vi "LabVIEW.Service.Create a failed report text from the report array.vi"(8 "error in (no error)":errorcluster caption="Fehler (Eingang, kein Fehler)", 11 "Result[[]]":string[][](array[string])) -> (0 "error out":errorcluster caption="Fehler (Ausgang)", 2 "Passed?":bool, 3 "report text":string)   [LabVIEW 2019]
uses:
  <userlib>/_OpenG.lib/array/array.llb/Search 1D Array (String)__ogtk.vi
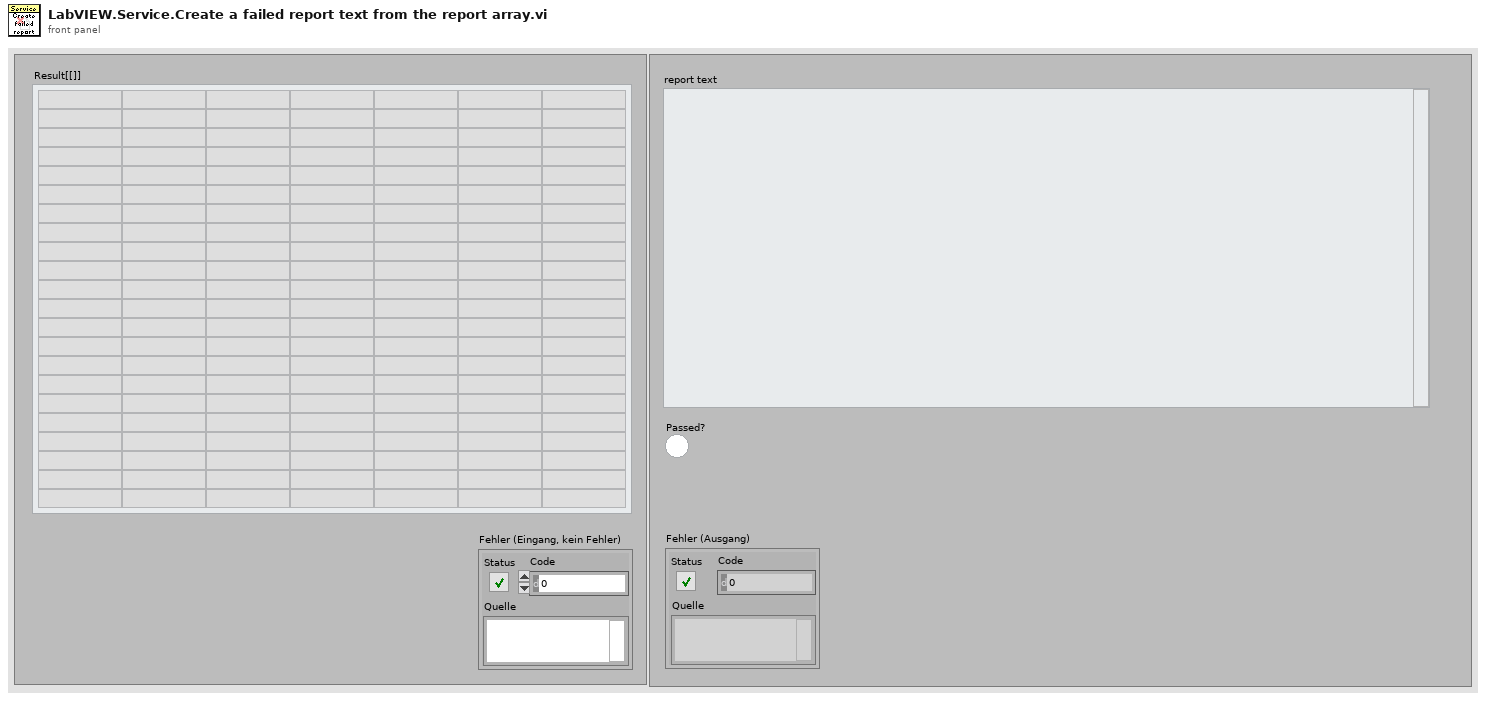
[diagram p1: front panel]
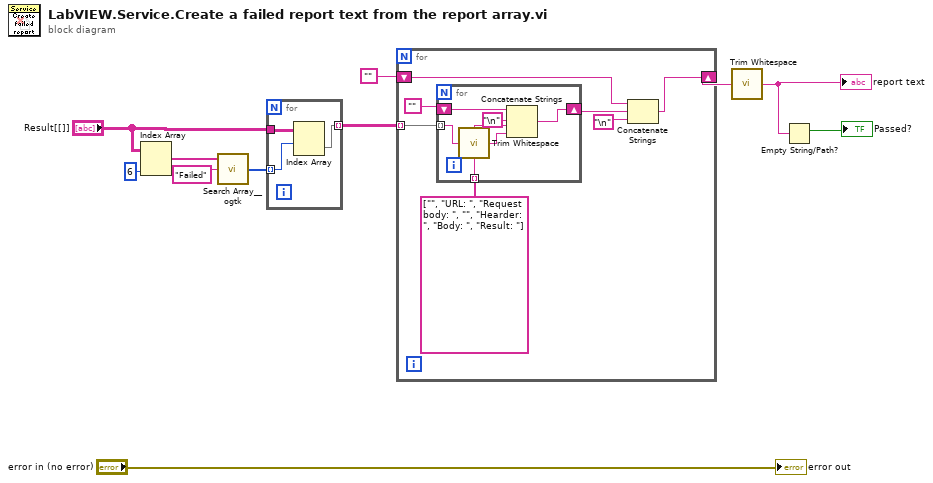
[diagram p0: block diagram]
diagram:
  n1 = Index Array(array="Result[[]]", index (col)=6 ("Deaktivierter Index (Spalte)")) -> (element=w9:string[])  [unwired: 1 in]
  n2 = call-poly <userlib>:"Search Array__ogtk.vi"("Array"=w9, "Element Data"="Failed") -> ("Indices of Elements"=w6:i32[])  [unwired: 7 in]
  n3 = for {
    tunnel: "Result[[]]" -> [w14]
    tunnel: w6 -> [w13] mode=indexing
    tunnel: [w12] -> w5 mode=indexing
    n4 = Index Array(array=w14, index (row)=w13) -> (element=w12:string[])  [unwired: 1 in]
  }
  n5 = for {
    tunnel: w5 -> [w21] mode=indexing
    shift-right: [w19] -> w4
    shift-left: "" -> [w18]
    n6 = for {
      tunnel: w21 -> [w22] mode=indexing
      shift-right: [w27] -> w20
      shift-left: "" -> [w26]
      tunnel: string[] ["", "URL: ", "Request body: ", "", "Hearder: ", "Body: ", "Result: "] -> [w24] mode=indexing
      n7 = call <vilib>:"Trim Whitespace.vi"("string"=w22) -> ("trimmed string"=w23:string)  [unwired: 1 in]
      n8 = Concatenate Strings(w26, "\n", w24, w23) -> (w27:string)
    }
    n9 = Concatenate Strings(w18, w20, "\n") -> (w19:string)
  }
  n10 = call <vilib>:"Trim Whitespace.vi"("string"=w4) -> ("trimmed string"=w2:string)  [unwired: 1 in]
  "report text" <- w2
  n11 = Empty String/Path?(string/path=w2) -> (empty?=→"Passed?":bool)
  "error out" <- "error in (no error)"
